vi "VIH Project - Verify CSS,JS,Template Files.vi"() -> (0 "error":bool, 1 "Message":string, 2 "Bad files":path[](array[path]))   [LabVIEW 2014]
doc: "::: VI Helpeks :::\nCopyright (c) 2000-2026 Konstantin Shifershteyn. All rights reserved."
panel:
  # "VI Helpeks\nCopyright (c) 2012-2026 Konstantin Shifershteyn"
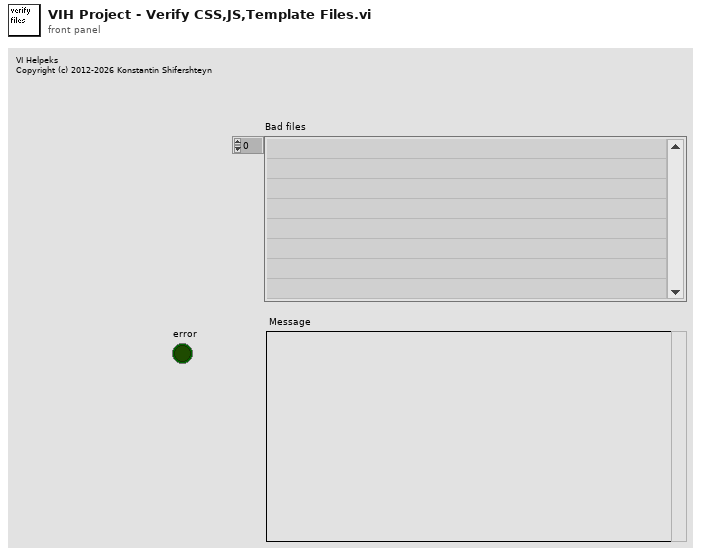
[diagram p1: front panel]
types:
  T1 = enum16{"get", "get all", "set", "Init", "delete", "rename"}
  T2 = enum16{"get", "get all", "set", "Init", "delete"}
  T3 = typedef "VIH HelpGen Typedef - Cluster - Group Rule.ctl" = cluster{"Source Root Dir":path, "Build Root Dir":path, "BuildHelp":T4, "Source Paths":T5, "Target Paths":T6, "VIDscrMode":T7, "MenuDscrMode":T7, "MenuItemIcons":T4, "Control Rules":T8[], "Flags":T10, "Ctl_DscrMode":T7, "Ctl_ClustMembers":T4, "Ctl_EnumValues":T4, "%Comments":string, "PVIIDscrMode":T7, "VIDetailsMode":T7, "ProductInfoMode":T4, "ProductInfoText":string}
  T4 = typedef "VIH HelpGen Typedef - Enum - Default,Enable,Disable.ctl" = enum16{"Default", "Enable", "Disable"}
  T5 = typedef "VIH HelpGen Typedef - Cluster - Group Rule - Source Paths.ctl" = cluster{"CSS Files":path[], "JS Files":path[], "VI Template":path, "Menu Template":path, "PolyVI Template":path}
  T6 = typedef "VIH HelpGen Typedef - Cluster - Group Rule - Target Paths.ctl" = cluster{"HTML Dir":path, "Image Dir":path, "CSS Dir":path, "JS Dir":path}
  T7 = typedef "VIH HelpGen Typedef - Enum - Description Mode.ctl" = enum16{"Default", "Description", "Description1", "Description2", "Custom", "None"}
  T8 = typedef "VIH HelpGen Typedef - Cluster - Control Rule.ctl" = cluster{"CtrlID":string, "CustomRule":bool, "DscrMode":T7, "Description":string, "ClusterMembers":T4, "EnumValues":T4, "EnumValDscr":T9[], "CustomName":string}
  T9 = typedef "VIH HelpGen Typedef - Cluster - Enum Value Info.ctl" = cluster{"Value":ext, "String":string, "Description":string}
  T10 = typedef "VIH HelpGen Typedef - Cluster - Group Rule - Flags.ctl" = cluster{"Override CSS Files":bool, "Override JS Files":bool, "Override Ctl Rules":bool}
  T11 = typedef "VIH HelpGen Typedef - Cluster - File Rule.ctl" = cluster{"OutName":string, "BuildHelp":T4, "Source Paths":T12, "Target Paths":T13, "DscrMode":T7, "Description":string, "Control Rules":T8[], "Flags":T10, "Ctl_DscrMode":T7, "Ctl_ClustMembers":T4, "Ctl_EnumValues":T4, "MenuItemIcons":T4, "%Comments":string, "DetailsMode":T7, "DetailsText":string, "ProductInfoMode":T4, "ProductInfoText":string}
  T12 = typedef "VIH HelpGen Typedef - Cluster - File Rule - Source Paths.ctl" = cluster{"CSS Files":path[], "JS Files":path[], "Html Template":path}
  T13 = typedef "VIH HelpGen Typedef - Cluster - File Rule - Target Paths.ctl" = cluster{"HTML Dir":path, "Image Dir":path, "CSS Dir":path, "JS Dir":path}
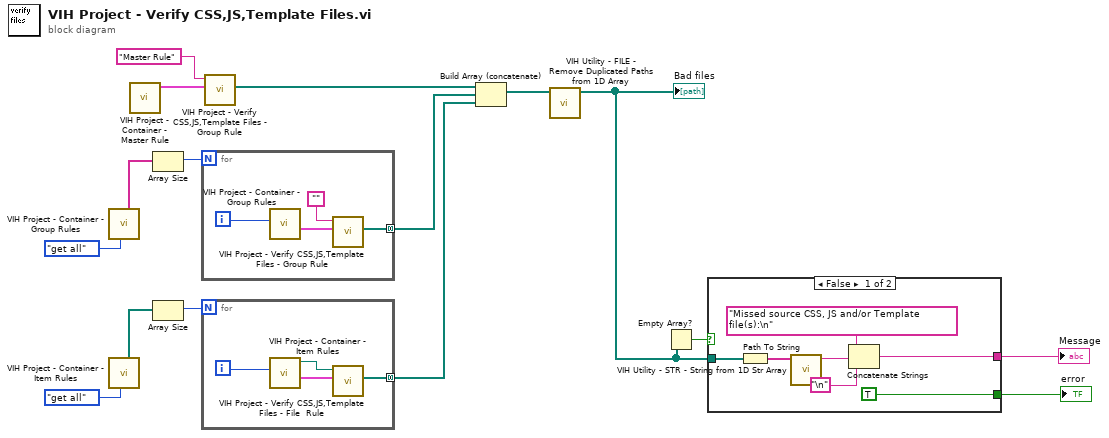
[diagram p0: block diagram]
diagram:
  n1 = call "VIH Project - Container - Group Rules.vi"("cmd (get)"=T2."get all") -> ("Group IDs"=w15:string[])  [unwired: 6 in, 4 out]
  n2 = call "VIH Project - Container - Item Rules.vi"("cmd (get)"=T1."get all") -> ("Item Paths"=w12:path[])  [unwired: 6 in, 4 out]
  n3 = call "VIH Project - Container - Master Rule.vi"() -> ("Rule out"=w10:T3)  [unwired: 11 in]
  n4 = Array Size(array=w15) -> (size(s)=w14:i32)
  n5 = Array Size(array=w12) -> (size(s)=w13:i32)
  n6 = for {
    N: w14 -> [_]
    tunnel: [w18] -> w7 mode=concatenating
    i -> [w20]
    n7 = call "VIH Project - Container - Group Rules.vi"("Group Idx (-1)"=w20) -> ("Group Rule out"=w19:T3)  [unwired: 6 in, 4 out]
    n8 = call "VIH Project - Verify CSS,JS,Template Files - Group Rule.vi"("Group Rule"=w19, "Group name"="") -> ("Bad files"=w18:path[])  [unwired: 9 in]
  }
  n9 = for {
    N: w13 -> [_]
    tunnel: [w24] -> w6 mode=concatenating
    i -> [w23]
    n10 = call "VIH Project - Container - Item Rules.vi"("Item Idx (-1)"=w23) -> ("Item Rule out"=w22:T11, "Item Path out"=w21:path)  [unwired: 6 in, 3 out]
    n11 = call "VIH Project - Verify CSS,JS,Template Files - File  Rule.vi"("File Rule"=w22, "File path"=w21) -> ("Bad files"=w24:path[])  [unwired: 9 in]
  }
  n12 = call "VIH Project - Verify CSS,JS,Template Files - Group Rule.vi"("Group Rule"=w10, "Group name"="Master Rule") -> ("Bad files"=w8:path[])  [unwired: 9 in]
  n13 = Build Array (concatenate)(w8, w7, w6) -> (w5:path[])
  n14 = call "VIH Utility - FILE - Remove Duplicated Paths from 1D Array.vi"("Array in"=w5) -> ("Array out"=w3:path[])  [unwired: 9 in, 1 out]
  "Bad files" <- w3
  n15 = Empty Array?(array=w3) -> (empty?=w4:bool)
  n16 = case shown="False" w4 {
    tunnel: w3 -> [w31 _]
    tunnel: [w27 _] -> w2
    tunnel: [TRUE _] -> w1
    frame False {
      n17 = Path To String(path=w31) -> (string=w30:string[])
      n18 = call "VIH Utility - STR - String from 1D Str Array.vi"("Array in"=w30) -> ("String out"=w29:string)  [unwired: 6 in]
      n19 = Concatenate Strings("Missed source CSS, JS and/or Template file(s):\n", w29, "\n") -> (w27:string)
    }
    frame True {
    }
  }
  "Message" <- w2
  "error" <- w1
